vi "Main Page.vi"(8 "error in (no error)":errorcluster, 11 "Node Ptr":T1 format="%.0x") -> (0 "error out":errorcluster)   [LabVIEW 2019, in "FPGA Addon System Explorer.lvlib"]
uses:
  FPGA Addon System Explorer.lvlib
  <vilib>/NI VeriStand/Custom Device API/Custom Device Item Ref.ctl
  Addon Shared/Types/FG Action.ctl
  <vilib>/NI/NI VeriStand Hardware Resource Discovery/_Types/Filter Type.ctl
  Addon Shared/SubVIs/Constants.vi
  <vilib>/NI VeriStand/Custom Device API/NI VeriStand - Get Item Property.vi
  <vilib>/NI VeriStand/Custom Device API/Get Item Property (Path).vi
  <vilib>/NI VeriStand/Custom Device API/Get Item Property (String).vi
  <vilib>/NI VeriStand/Custom Device API/Get Item Property (Boolean).vi
  <vilib>/NI VeriStand/Custom Device API/NI VeriStand - Set Item Property.vi
  <vilib>/NI VeriStand/Custom Device API/Set Item Property (Path).vi
  <vilib>/NI VeriStand/Custom Device API/Set Item Property (String).vi
  <vilib>/NI VeriStand/Custom Device API/Set Item Property (Boolean).vi
  <vilib>/NI VeriStand/Custom Device API/Custom Device API.lvlib
  Addon Shared/FPGA Addon Shared.lvlib
  <vilib>/NI/NI VeriStand Hardware Resource Discovery/NIVS Hardware Discovery.lvlib
panel:
  out "Group?":bool
  in  "RIO Browse":bool
  out "Version":string
  in  "SHDocVw.IWebBrowser":refnum<k7>(container)
  in  "RIO Device":string
  in  "Bitfile path":path
  in  "Header 2":cluster{"Section Name":string}={"Section Name"="FPGA Settings"}
  in  "Header":cluster{"Section Name":string}={"Section Name"="Addon Settings"}
  in  "Description":string
  in  "Name":string
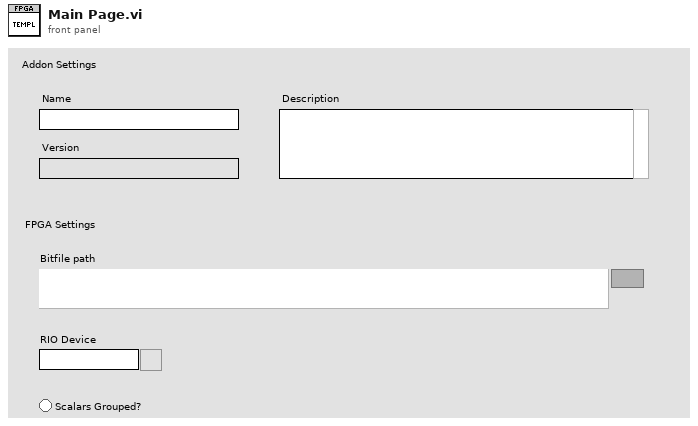
[diagram p1: front panel]
types:
  T1 = typedef "Custom Device API.lvlib/Custom Device Item Ref.ctl" = u64
  T2 = typedef "FPGA Addon Shared.lvlib/FG Action.ctl" = enum8{"GET", "SET"}
  T3 = typedef "FPGA Addon Shared.lvlib/FPGA Settings.ctl" = cluster{"Bitfile path":path, "RIO Device Address":string, "Group":bool}
  T4 = typedef "Custom Device API.lvlib/Custom Device Item Info.ctl" = cluster{"Name":string, "Is Channel":bool, "GUID":string, "Is Waveform":bool}
  T5 = typedef "NIVS Hardware Discovery.lvlib/Filter Type.ctl" = enum16{"Device Category", "Product Name", "Ethernet", "XNET", "VISA", "FPGA", "EtherCAT Master", "DAQmx", "GPIB", "Serial"}
  T6 = typedef "Custom Device API.lvlib/Custom Device Commands.ctl" = enum16{"Default", "Item renamed", "Shutdown", "Dynamic button pressed"}
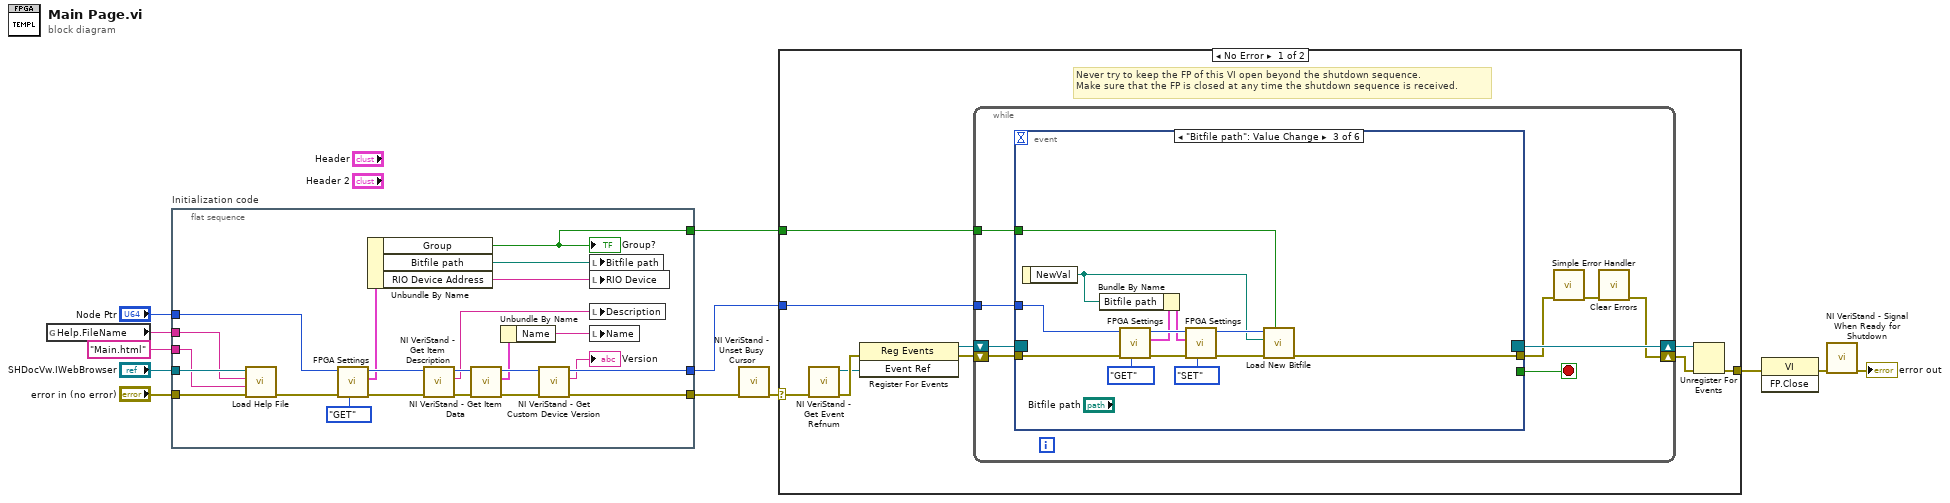
[diagram p0: block diagram]
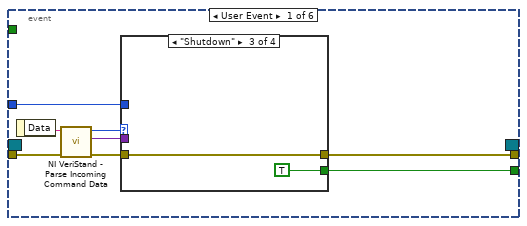
[diagram p2: hidden frame]
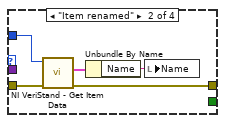
[diagram p4: hidden frame]
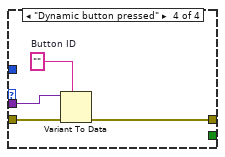
[diagram p5: hidden frame]
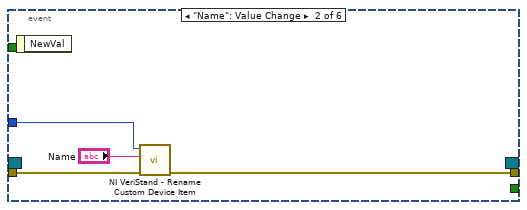
[diagram p6: hidden frame]
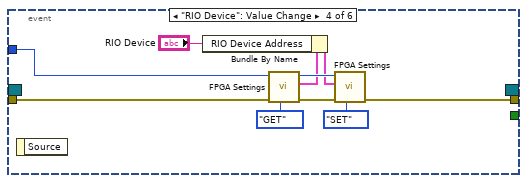
[diagram p7: hidden frame]
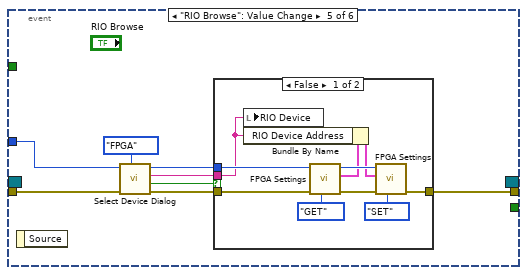
[diagram p8: hidden frame]
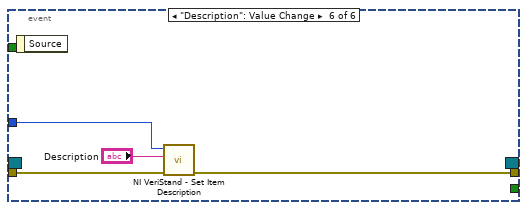
[diagram p10: hidden frame]
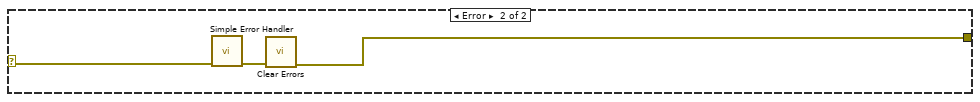
[diagram p11: hidden frame]
diagram:
  n1 = global read "Constants.vi" "Help.FileName"() -> (w2:string)
  n2 = flat-sequence "Initialization code" {
    tunnel: "error in (no error)" -> [w29]
    tunnel: "Node Ptr" -> [w25]
    tunnel: [w16] -> w8
    tunnel: [w17] -> w5
    tunnel: "SHDocVw.IWebBrowser" -> [w28]
    tunnel: "Main.html" ("HTML File") -> [w27]
    tunnel: w2 -> [w26]
    tunnel: [w13] -> w1
    frame #0 {
      n3 = call "Load Help File.vi"("error in (no error)"=w29, "HTML File"=w27, "Main CHM File"=w26, "SHDocVw.IWebBrowser2"=w28) -> ("error out"=w24:errorcluster)  [unwired: 7 in]
      n4 = call "FPGA Settings.vi"("Action"=FG_Action."GET", "error in (no error)"=w24, "Item Ref"=w25) -> ("error out"=w22:errorcluster, "FPGA Settings"=w20:T3, "Item Ref out"=w23:T1)  [unwired: 6 in]
      n5 = Unbundle By Name(w20) -> ("Group"=w13:bool, "Bitfile path"=w18:path, "RIO Device Address"=w19:string)
      "Group?" <- w13
      n6 = call <vilib>:"NI VeriStand - Get Item Description.vi"("error in (no error)"=w22, "Item Ref in"=w23) -> ("error out"=w32:errorcluster, "Description"=w33:string, "Item Ref out"=w34:T1)  [unwired: 7 out]
      n7 = call <vilib>:"NI VeriStand - Get Item Data.vi"("error in (no error)"=w32, "Item Ref in"=w34) -> ("error out"=w15:errorcluster, "Item Info"=w31:T4, "Item Ref out"=w35:T1)  [unwired: 7 out]
      n8 = Unbundle By Name(w31) -> ("Name"=w30:string)
      n9 = call <vilib>:"NI VeriStand - Get Custom Device Version.vi"("error in (no error)"=w15, "Device Ref in"=w35) -> ("error out"=w16:errorcluster, "Value"=→"Version":string, "Device Ref out"=w17:T1)  [unwired: 7 in]
      n10 = local write "Bitfile path"(w18) -> ()
      n11 = local write "RIO Device"(w19) -> ()
      n12 = local write "Description"(w33) -> ()
      n13 = local write "Name"(w30) -> ()
    }
  }
  n14 = call <vilib>:"NI VeriStand - Unset Busy Cursor.vi"("error in (no error)"=w8) -> ("error out"=w7:errorcluster)  [unwired: 10 out]
  n15 = case shown="No Error" w7 {
    selector: w7 -> [w37 w127]
    tunnel: [w42 w125] -> w12
    tunnel: w5 -> [w38 _]
    tunnel: w1 -> [w36 _]
    frame No Error {
      # "Never try to keep the FP of this VI open beyond the shutdown sequence.\nMake sure that the FP is closed at any time the shutdown sequence is received."
      n16 = call <vilib>:"NI VeriStand - Get Event Refnum.vi"("error in (no error)"=w37) -> ("error out"=w45:errorcluster, "Event Ref"=w41:refnum<user-event>)  [unwired: 9 out]
      n17 = register-events(error in=w45, w41) -> (reference out=w39:refnum<event-registration>, error out=w40:errorcluster)  [unwired: 1 in]
      n18 = while {
        tunnel: w38 -> [w50]
        shift-right: [w47] -> w43
        shift-left: w40 -> [w53]
        shift-right: [w54] -> w44
        shift-left: w39 -> [w52]
        tunnel: w36 -> [w46]
        stop <- w51 stop-if-true
        n19 = event shown="[2] \"Bitfile path\": Value Change" {
          selector: w52 -> [_ _ _ _ _ _]
          dyn-events: [_ _ _ _ _ _] -> w54
          timeout: _ -> [_ _ _ _ _ _]
          tunnel: w53 -> [w62 w78 w86 w95 w107 w123]
          tunnel: [w58 _ _ _ _ _] -> w51
          tunnel: [w57 w77 w91 w92 w109 w122] -> w49
          tunnel: w50 -> [w56 w76 w84 w94 w108 w124]
          tunnel: w46 -> [_ _ w79 _ _ _]
          event User Event {
            n20 = event-data() -> ("Data"=w61:string)  [unwired: 1 out]
            n21 = call <vilib>:"NI VeriStand - Parse Incoming Command Data.vi"("error in (no error)"=w62, "Incoming data"=w61) -> ("error out"=w60:errorcluster, "Outgoing data"=w55:variant, "Action"=w59:T6)  [unwired: 7 out]
            n22 = case shown="\"Shutdown\"" w59 {
              tunnel: w60 -> [w63 w68 w69 w74]
              tunnel: [_ _ TRUE _] -> w58
              tunnel: [w63 w65 w69 w71] -> w57
              tunnel: w56 -> [_ w67 _ _]
              tunnel: w55 -> [_ _ _ w73]
              frame "Default", Default {
              }
              frame "Item renamed" {
                n23 = call <vilib>:"NI VeriStand - Get Item Data.vi"("error in (no error)"=w68, "Item Ref in"=w67) -> ("error out"=w65:errorcluster, "Item Info"=w66:T4)  [unwired: 8 out]
                n24 = Unbundle By Name(w66) -> ("Name"=w64:string)
                n25 = local write "Name"(w64) -> ()
              }
              frame "Shutdown" {
              }
              frame "Dynamic button pressed" {
                w72 = ""  # Button ID
                n26 = Variant To Data(error in=w74, type=w72, Variant=w73) -> (error out=w71:errorcluster)  [unwired: 1 out]
              }
            }
          }
          event "Name": Value Change {
            n27 = event-data() -> ()  [unwired: 2 out]
            n28 = call <vilib>:"NI VeriStand - Rename Custom Device Item.vi"("error in (no error)"=w78, "New Name"="Name", "Item Ref in"=w76) -> ("error out"=w77:errorcluster)  [unwired: 1 in, 7 out]
          }
          event "Bitfile path": Value Change {
            n29 = event-data() -> ("NewVal"=w80:path)  [unwired: 1 out]
            n30 = call "FPGA Settings.vi"("Action"=FG_Action."GET", "error in (no error)"=w86, "Item Ref"=w84) -> ("error out"=w87:errorcluster, "FPGA Settings"=w82:T3, "Item Ref out"=w88:T1)  [unwired: 6 in]
            n31 = Bundle By Name(cluster=w82, "Bitfile path"=w80) -> (w81:T3)
            n32 = call "FPGA Settings.vi"("Action"=FG_Action."SET", "error in (no error)"=w87, "FPGA Settings"=w81, "Item Ref"=w88) -> ("error out"=w85:errorcluster, "Item Ref out"=w83:T1)  [unwired: 5 in, 1 out]
            n33 = call "Load New Bitfile.vi"("Group"=w79, "error in (no error)"=w85, "NewVal"=w80, "Item Ref in"=w83) -> ("error out"=w91:errorcluster)  [unwired: 6 in, 1 out]
          }
          event "RIO Device": Value Change {
            n34 = event-data() -> ()  [unwired: 2 out]
            n35 = call "FPGA Settings.vi"("Action"=FG_Action."GET", "error in (no error)"=w95, "Item Ref"=w94) -> ("error out"=w98:errorcluster, "FPGA Settings"=w97:T3, "Item Ref out"=w99:T1)  [unwired: 6 in]
            n36 = Bundle By Name(cluster=w97, "RIO Device Address"="RIO Device") -> (w96:T3)
            n37 = call "FPGA Settings.vi"("Action"=FG_Action."SET", "error in (no error)"=w98, "FPGA Settings"=w96, "Item Ref"=w99) -> ("error out"=w92:errorcluster)  [unwired: 5 in, 2 out]
          }
          event "RIO Browse": Value Change {
            n38 = event-data() -> ()  [unwired: 2 out]
            n39 = call <vilib>:"Select Device Dialog.vi"("Filter Type"=Filter_Type."FPGA", "error in (no error)"=w107, "Item Ref in"=w108) -> ("error out"=w105:errorcluster, "Cancelled?"=w104:bool, "Selected Alias"=w103:string, "Item Ref out"=w106:T1)  [unwired: 5 in]
            n40 = case shown="False" w104 {
              tunnel: w105 -> [w113 w120]
              tunnel: w106 -> [w112 _]
              tunnel: [w111 w120] -> w109
              tunnel: w103 -> [w110 _]
              frame False {
                n41 = local write "RIO Device"(w110) -> ()
                n42 = call "FPGA Settings.vi"("Action"=FG_Action."GET", "error in (no error)"=w113, "Item Ref"=w112) -> ("error out"=w116:errorcluster, "FPGA Settings"=w115:T3, "Item Ref out"=w117:T1)  [unwired: 6 in]
                n43 = Bundle By Name(cluster=w115, "RIO Device Address"=w110) -> (w114:T3)
                n44 = call "FPGA Settings.vi"("Action"=FG_Action."SET", "error in (no error)"=w116, "FPGA Settings"=w114, "Item Ref"=w117) -> ("error out"=w111:errorcluster)  [unwired: 5 in, 2 out]
              }
              frame True {
              }
            }
          }
          event "Description": Value Change {
            n45 = event-data() -> ()  [unwired: 2 out]
            n46 = call <vilib>:"NI VeriStand - Set Item Description.vi"("error in (no error)"=w123, "Description"="Description", "Item Ref in"=w124) -> ("error out"=w122:errorcluster)  [unwired: 8 out]
          }
        }
        n47 = call <vilib>:"Simple Error Handler.vi"("error in (no error)"=w49) -> ("error out"=w48:errorcluster)  [unwired: 1 in, 7 out]
        n48 = call <vilib>:"Clear Errors.vi"("error in (no error)"=w48) -> ("error out"=w47:errorcluster)  [unwired: 1 in, 5 out]
      }
      n49 = Unregister For Events(event registration refnum=w44, error in=w43) -> (error out=w42:errorcluster)
    }
    frame Error {
      n50 = call <vilib>:"Simple Error Handler.vi"("error in (no error)"=w127) -> ("error out"=w126:errorcluster)  [unwired: 1 in, 7 out]
      n51 = call <vilib>:"Clear Errors.vi"("error in (no error)"=w126) -> ("error out"=w125:errorcluster)  [unwired: 1 in, 5 out]
    }
  }
  n52 = invoke class="VI" method="FP.Close"(error in=w12) -> (error out=w11:errorcluster)  [unwired: 2 in, 2 out]
  n53 = call <vilib>:"NI VeriStand - Signal When Ready for Shutdown.vi"("error in (no error)"=w11) -> ("error out"=→"error out":errorcluster)  [unwired: 10 out]
